vi "Launch Configured Tasks.vi"(8 "error in (no error)":errorcluster, 11 "Volatus Core in":refnum<class "Volatus Core.lvclass">) -> (0 "error out":errorcluster, 3 "Volatus Core out":refnum<class "Volatus Core.lvclass">)   [LabVIEW 2020, in "Volatus.lvlib" / "Volatus Core.lvclass"]
uses:
  Volatus Core.lvclass
  C:/dev/lv20CE/relink/lv-volatus/Volatus/Module/Module.lvclass
  Volatus Core.lvclass/Volatus Core.ctl
  Module/Module.lvclass/Module.ctl
  VolatusConfig/Task/Task Config.lvclass
  C:/dev/lv20CE/relink/lv-volatus/VolatusConfig/VolatusConfigElement/VolatusConfigElement.lvclass
  MessageQ/MessageQ.lvclass
  Module/Module.lvclass
  VolatusAPI/VolatusAPI.lvclass
  VolatusConfig/Node/Node Config.lvclass
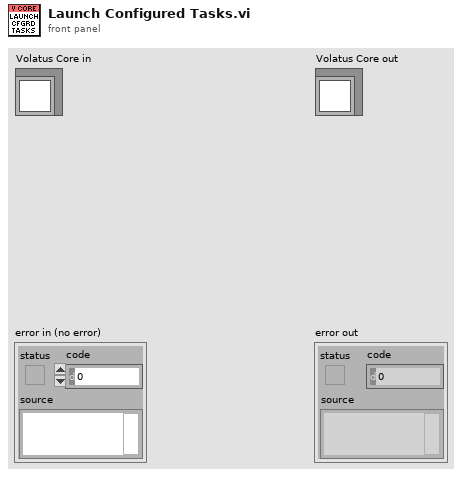
[diagram p1: front panel]
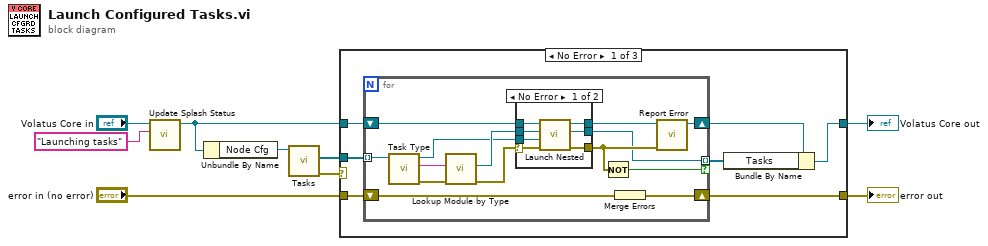
[diagram p0: block diagram]
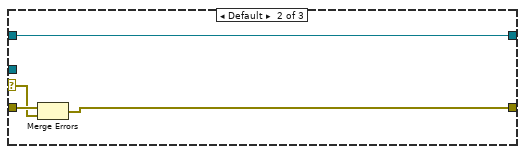
[diagram p3: hidden frame]
diagram:
  n1 = call "Update Splash Status.vi"("Status"="Launching tasks", "Volatus Core in"="Volatus Core in") -> ("Volatus Core out"=w2:refnum<class "Volatus Core.lvclass">)  [unwired: 8 in, 1 out]
  n2 = Unbundle By Name(w2) -> ("Node Cfg"=w8:refnum<class "Node Config.lvclass">)
  n3 = call "Tasks.vi"("Node in"=w8) -> ("error out"=w3:errorcluster, "Tasks"=w7:refnum<class "Task Config.lvclass">[])  [unwired: 8 in, 1 out]
  n4 = case shown="No Error" w3 {
    selector: w3 -> [_ w41 _]
    tunnel: [w16 w40 w45] -> w9
    tunnel: w7 -> [w14 _ _]
    tunnel: "error in (no error)" -> [w13 w42 w45]
    tunnel: w2 -> [w12 w43 w44]
    tunnel: [w11 w43 w44] -> w4
    frame No Error {
      n5 = for {
        tunnel: w14 -> [w23] mode=indexing
        shift-right: [w17] -> w15
        shift-left: w12 -> [w29]
        shift-right: [w24] -> w16
        shift-left: w13 -> [w25]
        tunnel: [w19] -> w10 mode=indexing if=w18
        n6 = call "Task Type.vi"("Task in"=w23) -> ("error out"=w20:errorcluster, "Task Type"=w21:string, "Task out"=w22:refnum<class "Task Config.lvclass">)  [unwired: 8 in]
        n7 = call "Lookup Module by Type.vi"("error in (no error)"=w20, "Module Type"=w21) -> ("error out"=w27:errorcluster, "Module Type"=w28:refnum<class "Module.lvclass">)  [unwired: 8 in]
        n8 = case shown="No Error" w27 {
          selector: w27 -> [w34 w38]
          tunnel: w29 -> [w37 w39]
          tunnel: w28 -> [w36 _]
          tunnel: w22 -> [w35 _]
          tunnel: [w33 w38] -> w30
          tunnel: [w32 w39] -> w26
          tunnel: [w31 _] -> w19
          frame No Error {
            n9 = call "Launch Nested.vi"("error in (no error)"=w34, "Config Element"=w35, "Nested Module"=w36, "Parent in"=w37) -> ("error out"=w33:errorcluster, "MessageQ"=w31:refnum<class "MessageQ.lvclass">, "Parent out"=w32:refnum<class "Volatus Core.lvclass">)  [unwired: 5 in]
          }
          frame Error {
          }
        }
        n10 = Not(x=w30) -> (.not. x?=w18:bool)
        n11 = Merge Errors(w25) -> (w24:errorcluster)
        n12 = call "Report Error.vi"("error in (no error)"=w30, "Module in"=w26) -> ("Module out"=w17:refnum<class "Volatus Core.lvclass">)  [unwired: 8 in, 1 out]
      }
      n13 = Bundle By Name(cluster=w15, "Tasks"=w10) -> (w11:refnum<class "Volatus Core.lvclass">)
    }
    frame Default {
      n14 = Merge Errors(w42, w41) -> (w40:errorcluster)
    }
    frame Error {
      # "Tasks entry not present, this can be the case for command server apps, though eventually those will have a status GUI. Also for unconfigured systems."
    }
  }
  "error out" <- w9
  "Volatus Core out" <- w4
